vi "Connect.vi"(8 "error in (no error)":errorcluster, 11 "Modbus in":refnum<class "Modbus.lvclass">) -> (0 "error out":errorcluster, 3 "Modbus out":refnum<class "Modbus.lvclass">)   [LabVIEW 2026, in "Modbus.lvlib" / "Modbus.lvclass"]
uses:
  Modbus.lvclass
  Modbus.lvclass/Modbus.ctl
  <vilib>/NI/Modbus Library/API/Wrapper/Create TCP Master.vi
  <vilib>/NI/Modbus Library/API/Wrapper/API Main.lvlib
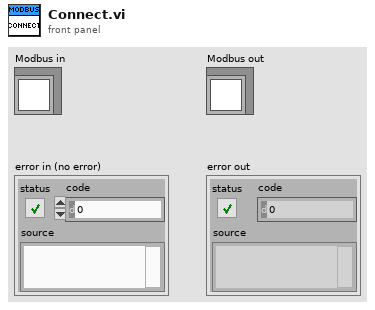
[diagram p1: front panel]
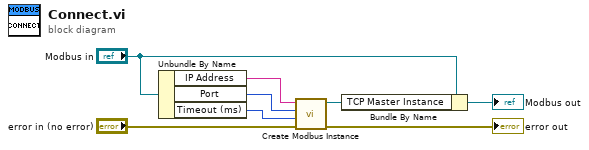
[diagram p0: block diagram]
diagram:
  n1 = Unbundle By Name("Modbus in") -> ("IP Address"=w5:string, "Port"=w6:u16, "Timeout (ms)"=w7:i32)
  n2 = call-poly <vilib>:"Create Modbus Instance.vi"("error in"="error in (no error)", "connect timeout ms"=w7, "port (502)"=w6, "address"=w5) -> ("error out"=→"error out":errorcluster, "TCP master instance"=w3:refnum<class "Modbus Master.lvclass">)  [unwired: 6 in]
  n3 = Bundle By Name(cluster="Modbus in", "TCP Master Instance"=w3) -> (→"Modbus out":refnum<class "Modbus.lvclass">)
